vi "FuncVI-FileBuildPath.vi"(5 "InstanceRef":T2, 9 "arg list":T1[](array[typedef]) {"num" format="%.2f"}) -> (0 "error out":bool, 3 "result":T1 {"num" format="%.2f"})   [LabVIEW 2021]
doc: "::: CalcExpress Toolkit :::\nCopyright (c) 2000-2026 Konstantin Shifershteyn. All rights reserved."
uses:
  cetypes.llb/CalcExpress Function Argument Info.ctl
  cetypes.llb/CalcExpress Instance RefNum.ctl
panel:
  in  "max arg num":i32=1000
  in  "min arg num":i32=1
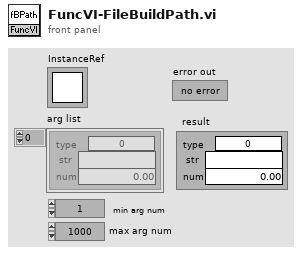
[diagram p1: front panel]
types:
  T1 = typedef "CalcExpress Function Argument Info.ctl" = cluster{"type":u32, "str":string, "num":dbl}
  T2 = typedef "CalcExpress Instance RefNum.ctl" = refnum<k1>
  T3 = enum32{"String", "DBL Number", "identifier", "1D Array of DBL", "2D Array of DBL", "CDB Number", "1D Array of CDB", "2D Array of CDB", "1D Array of String", "2D Array of String", "Unknown data type"}
  T4 = cluster{"type: use this constant to specify a predefined type code":enum32{"String", "DBL Number", "identifier", "1D Array of DBL", "2D Array of DBL", "CDB Number", "1D Array of CDB", "2D Array of CDB", "1D Array of String", "2D Array of String", "Unknown data type"}, string, dbl}
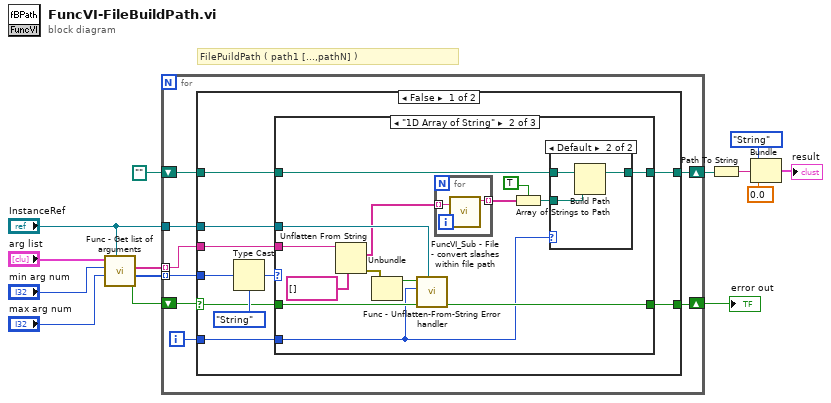
[diagram p0: block diagram]
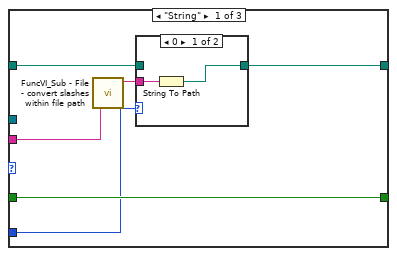
[diagram p2: hidden frame]
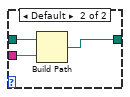
[diagram p3: hidden frame]
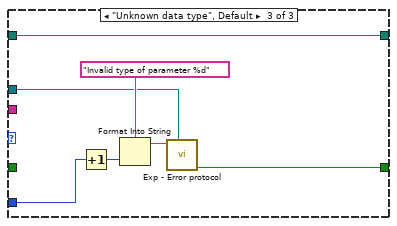
[diagram p5: hidden frame]
diagram:
  # "FilePuildPath ( path1 [...,pathN] )"
  n1 = call "Func - Get list of arguments.vi"("InstanceRef"="InstanceRef", "max arg num"="max arg num", "min arg num"="min arg num", "arg list"="arg list") -> ("error out"=w10:bool, "type list"=w9:u32[], "str list"=w8:string[])  [unwired: 4 in, 1 out]
  n2 = for {
    shift-right: [w20] -> w3
    shift-left: w10 -> [w21]
    tunnel: w9 -> [w22] mode=indexing
    tunnel: w8 -> [w19] mode=indexing
    tunnel: "InstanceRef" -> [w17]
    shift-right: [w15] -> w5
    shift-left: path "" -> [w16]
    i -> [w18]
    n3 = case shown="False" w21 {
      selector: w21 -> [w25 w72]
      tunnel: w22 -> [w32 _]
      tunnel: [w27 w72] -> w20
      tunnel: w19 -> [w29 _]
      tunnel: w18 -> [w28 _]
      tunnel: w17 -> [w26 _]
      tunnel: w16 -> [w24 w71]
      tunnel: [w23 w71] -> w15
      frame False {
        n4 = Type Cast(type=T3."String" ("type: use this constant to specify a predefined type code"), x=w32) -> (*(type *) &x=w31:T3)
        n5 = case shown="\"1D Array of String\"" w31 {
          tunnel: w29 -> [w33 w57 _]
          tunnel: w28 -> [w35 w48 w69]
          tunnel: [w38 w54 w66] -> w27
          tunnel: w26 -> [_ w53 w65]
          tunnel: w25 -> [w38 w55 _]
          tunnel: w24 -> [w37 w51 w64]
          tunnel: [w36 w50 w64] -> w23
          frame "String" {
            n6 = call "FuncVI_Sub - File - convert slashes within file path.vi"("str: path"=w33) -> ("str: path out"=w34:string)  [unwired: 3 in, 1 out]
            n7 = case shown="0" w35 {
              tunnel: w37 -> [_ w43]
              tunnel: w34 -> [w40 w42]
              tunnel: [w39 w41] -> w36
              frame 0 {
                n8 = String To Path(string=w40) -> (path=w39:path)
              }
              frame Default {
                n9 = Build Path(base path=w43, name or relative path=w42) -> (appended path=w41:path)
              }
            }
          }
          frame "1D Array of String" {
            n10 = Unflatten From String(type=string[] [] ("str list"), binary string=w57) -> (value=w45:string[], error out=w44:errorcluster)  [unwired: 3 in, 1 out]
            n11 = Unbundle(w44) -> ("status"=w52:bool)  [unwired: 2 out]
            n12 = call "Func - Unflatten-From-String Error handler.vi"("InstanceRef"=w53, "error in"=w55, "argument number"=w48, "Unflatten Error status"=w52) -> ("error out"=w54:bool)  [unwired: 5 in]
            n13 = for {
              tunnel: [w59] -> w46 mode=indexing
              tunnel: w45 -> [w58] mode=indexing
              n14 = call "FuncVI_Sub - File - convert slashes within file path.vi"("str: path"=w58) -> ("str: path out"=w59:string)  [unwired: 3 in, 1 out]
            }
            n15 = Array of Strings to Path(0:w46, 1:TRUE ("relative")) -> (2:w47:path)
            n16 = case shown="Default" w48 {
              tunnel: w51 -> [_ w63]
              tunnel: [w60 w62] -> w50
              tunnel: w47 -> [w60 w61]
              frame 0 {
              }
              frame Default {
                n17 = Build Path(base path=w63, name or relative path=w61) -> (appended path=w62:path)
              }
            }
          }
          frame "Unknown data type", Default {
            n18 = Increment(x=w69) -> (x+1=w68:i32)
            n19 = Format Into String(format string="Invalid type of parameter %d", w68) -> (resulting string=w67:string)  [unwired: 2 in, 1 out]
            n20 = call "Exp - Error protocol.vi"("InstanceRef"=w65, "error message in"=w67) -> ("error out"=w66:bool)  [unwired: 6 in, 1 out]
          }
        }
      }
      frame True {
      }
    }
  }
  "error out" <- w3
  n21 = Path To String(path=w5) -> (string=w4:string)
  n22 = Bundle("type: use this constant to specify a predefined type code"=T3."String", w4, 0.0) -> (→"result":T4)  [unwired: 1 in]
